vi "Obtain Request Events.vi"(8 "error in":errorcluster, 10 "Create New? (F)":bool) -> (0 "error out":errorcluster, 2 "Data Viewer Request Events":T1)   [LabVIEW 2020, in "Data Viewer.lvlib"]
doc: "This VI Obtains/Creates the Requests events that will be used for other modules to communicate with the module that owns this VI. These Requests events will be accessed only via Public API methods for this module.\n\n<b>NOTE</b>: The contents of this VI are automatically generated and modified by the <b>Tools > DQMH Consortium > DQMH</b> utilities. Consider using those utilities instead of making your own modifications to this VI.\n_____\nBased on DQMH Project Template 7.0.1.1316."
uses:
  Data Viewer.lvlib
  Request Events--cluster.ctl
  Stop Argument--cluster.ctl
  Show Panel Argument--cluster.ctl
  Hide Panel Argument--cluster.ctl
  Show Diagram Argument--cluster.ctl
  Get Module Execution Status Argument--cluster.ctl
  Window Resize Argument--cluster.ctl
  Open File Argument--cluster.ctl
  Draw Plot Argument--cluster.ctl
  Set YScale Argument--cluster.ctl
  Update Curve Color Argument--cluster.ctl
  Show Value Argument--cluster.ctl
  <vilib>/Utility/miscctls.llb/LVPoint32TypeDef.ctl
  Menu Action Argument--cluster.ctl
  Update Filter Arguments Argument--cluster.ctl
  Filte Data Argument--cluster.ctl
  Restore Data Argument--cluster.ctl
  Cut Half Data Argument--cluster.ctl
  Select Point Argument--cluster.ctl
  Open Linear Measurement Argument--cluster.ctl
  Linear Measurement Close Argument--cluster.ctl
  Scale List Menu Action Argument--cluster.ctl
  Update Scale List Argument--cluster.ctl
  Initialize Plot List Argument--cluster.ctl
  Load Plot Argument--cluster.ctl
  Unload Plot Argument--cluster.ctl
  Show Hide Scale Argument--cluster.ctl
  Add Default Scale Argument--cluster.ctl
  Update Plot List Argument--cluster.ctl
  Add Virtual Cruve Argument--cluster.ctl
  Edit Curve Argument--cluster.ctl
panel:
  # "NOTE: The contents of this VI are automatically generated and modified by the Tools > DQMH Consortium > DQMH utilities. Consider using those utilities instead of making your own modifications to this VI."
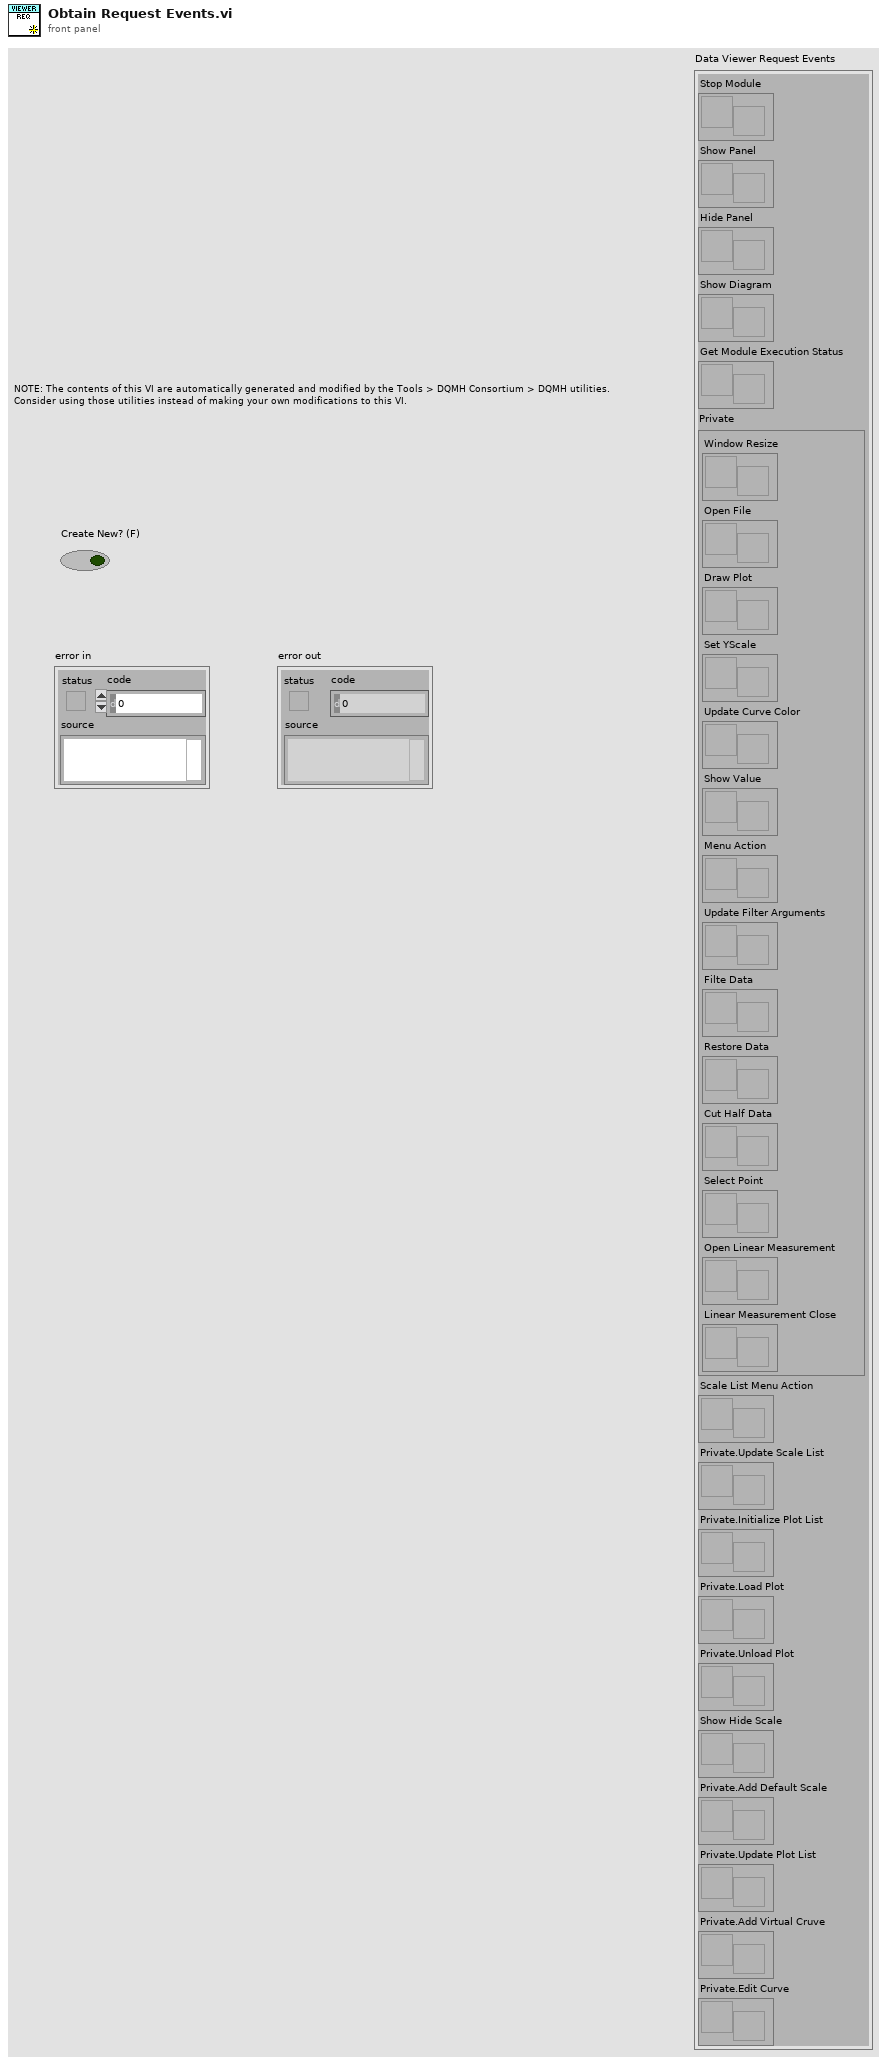
[diagram p1: front panel]
types:
  T1 = typedef "Data Viewer.lvlib/Request Events--cluster.ctl" = cluster{"Stop Module":refnum<user-event>, "Show Panel":refnum<user-event>, "Hide Panel":refnum<user-event>, "Show Diagram":refnum<user-event>, "Get Module Execution Status":refnum<user-event>, "Private":cluster{"Window Resize":refnum<user-event>, "Open File":refnum<user-event>, "Draw Plot":refnum<user-event>, "Set YScale":refnum<user-event>, "Update Curve Color":refnum<user-event>, "Show Value":refnum<user-event>, "Menu Action":refnum<user-event>, "Update Filter Arguments":refnum<user-event>, "Filte Data":refnum<user-event>, "Restore Data":refnum<user-event>, "Cut Half Data":refnum<user-event>, "Select Point":refnum<user-event>, "Open Linear Measurement":refnum<user-event>, "Linear Measurement Close":refnum<user-event>}, "Scale List Menu Action":refnum<user-event>, "Private.Update Scale List":refnum<user-event>, "Private.Initialize Plot List":refnum<user-event>, "Private.Load Plot":refnum<user-event>, "Private.Unload Plot":refnum<user-event>, "Show Hide Scale":refnum<user-event>, "Private.Add Default Scale":refnum<user-event>, "Private.Update Plot List":refnum<user-event>, "Private.Add Virtual Cruve":refnum<user-event>, "Private.Edit Curve":refnum<user-event>}
  T2 = typedef "Data Viewer.lvlib/Edit Curve Argument--cluster.ctl" = cluster{"Module ID":i32, "Plot Index":i32}
  T3 = typedef "Data Viewer.lvlib/Add Virtual Cruve Argument--cluster.ctl" = cluster{"Module ID":i32, "Boolean":bool}
  T4 = typedef "Data Viewer.lvlib/Update Plot List Argument--cluster.ctl" = cluster{"Module ID":i32, "曲线列表":cluster{"Name":string, "Scale":u16, "Color":u32, "Visible":bool, "Peak Line":bool}[]}
  T5 = typedef "Data Viewer.lvlib/Add Default Scale Argument--cluster.ctl" = cluster{"Module ID":i32, "Boolean":bool}
  T6 = typedef "Data Viewer.lvlib/Show Hide Scale Argument--cluster.ctl" = cluster{"Module ID":i32, "Scale Index":i32, "Visible":bool}
  T7 = typedef "Data Viewer.lvlib/Unload Plot Argument--cluster.ctl" = cluster{"Module ID":i32, "Plot Index":i32}
  T8 = typedef "Data Viewer.lvlib/Load Plot Argument--cluster.ctl" = cluster{"Module ID":i32, "Plot Index":i32}
  T9 = typedef "Data Viewer.lvlib/Initialize Plot List Argument--cluster.ctl" = cluster{"Module ID":i32, "Boolean":bool}
  T10 = typedef "Data Viewer.lvlib/Update Scale List Argument--cluster.ctl" = cluster{"Module ID":i32, "Boolean":bool}
  T11 = typedef "Data Viewer.lvlib/Scale List Menu Action Argument--cluster.ctl" = cluster{"Module ID":i32, "ItemTag ":string, "Scale Index":i32}
  T12 = typedef "Data Viewer.lvlib/Linear Measurement Close Argument--cluster.ctl" = cluster{"Module ID":i32, "Linear Measurement Module ID":i32}
  T13 = typedef "Data Viewer.lvlib/Open Linear Measurement Argument--cluster.ctl" = cluster{"Module ID":i32, "Linear Measurement Module ID":i32}
  T14 = typedef "Data Viewer.lvlib/Select Point Argument--cluster.ctl" = cluster{"Module ID":i32, "布尔":bool}
  T15 = typedef "Data Viewer.lvlib/Cut Half Data Argument--cluster.ctl" = cluster{"Module ID":i32, "布尔":bool}
  T16 = typedef "Data Viewer.lvlib/Restore Data Argument--cluster.ctl" = cluster{"Module ID":i32, "布尔":bool}
  T17 = typedef "Data Viewer.lvlib/Filte Data Argument--cluster.ctl" = cluster{"Module ID":i32, "布尔":bool}
  T18 = typedef "Data Viewer.lvlib/Update Filter Arguments Argument--cluster.ctl" = cluster{"Module ID":i32, "布尔":bool}
  T19 = typedef "Data Viewer.lvlib/Menu Action Argument--cluster.ctl" = cluster{"Module ID":i32, "项标识符":string}
  T20 = typedef "Data Viewer.lvlib/Show Value Argument--cluster.ctl" = cluster{"Module ID":i32, "坐标":T21}
  T21 = typedef "LVPoint32TypeDef.ctl" = cluster{"Horizontal":i32, "Vertical":i32}
  T22 = typedef "Data Viewer.lvlib/Update Curve Color Argument--cluster.ctl" = cluster{"Module ID":i32, "布尔":bool}
  T23 = typedef "Data Viewer.lvlib/Set YScale Argument--cluster.ctl" = cluster{"Module ID":i32, "布尔":bool}
  T24 = typedef "Data Viewer.lvlib/Draw Plot Argument--cluster.ctl" = cluster{"Module ID":i32, "布尔":bool}
  T25 = typedef "Data Viewer.lvlib/Open File Argument--cluster.ctl" = cluster{"Module ID":i32, "布尔":bool}
  T26 = typedef "Data Viewer.lvlib/Window Resize Argument--cluster.ctl" = cluster{"Module ID":i32, "布尔":bool}
  T27 = typedef "Data Viewer.lvlib/Get Module Execution Status Argument--cluster.ctl" = cluster{"Module ID":i32, "Running?":bool}
  T28 = typedef "Data Viewer.lvlib/Show Diagram Argument--cluster.ctl" = cluster{"Module ID":i32, "Debug?":bool}
  T29 = typedef "Data Viewer.lvlib/Show Panel Argument--cluster.ctl" = cluster{"Module ID":i32, "Show Panel?":bool}
  T30 = typedef "Data Viewer.lvlib/Hide Panel Argument--cluster.ctl" = cluster{"Module ID":i32, "Hide Panel?":bool}
  T31 = typedef "Data Viewer.lvlib/Stop Argument--cluster.ctl" = cluster{"Module ID":i32, "Origin":string, "Exit via Stop Module Req?":bool, "Wait for Module to stop?":bool}
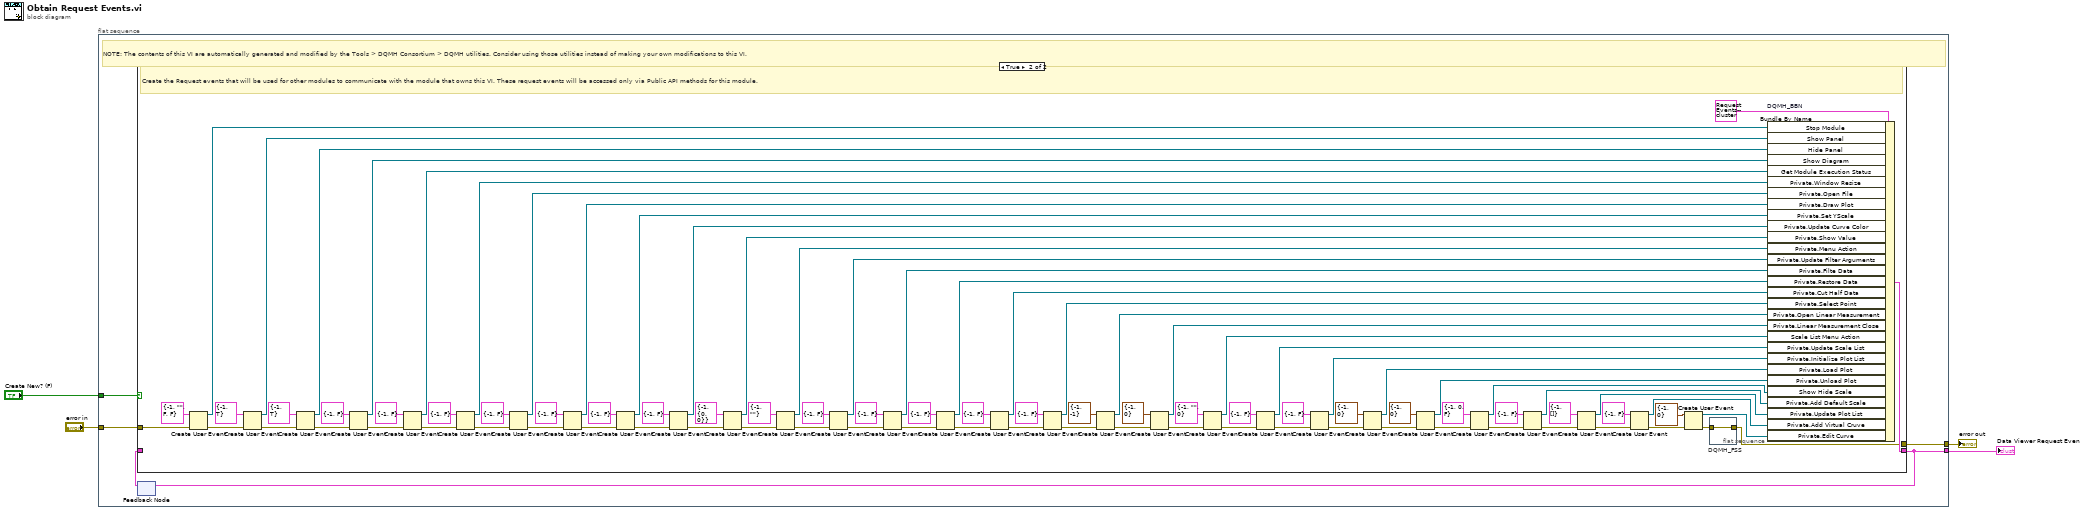
[diagram p0: block diagram]
diagram:
  n1 = flat-sequence {
    tunnel: [w9] -> w4
    tunnel: "error in" -> [w8]
    tunnel: [w6] -> w2
    tunnel: "Create New? (F)" -> [w5]
    frame #0 {
      # "NOTE: The contents of this VI are automatically generated and modified by the Tools > DQMH Consortium > DQMH utilities. Consider using those utilities instead of making your own modifications to this VI."
      n2 = feedback #1() -> (w7:T1)  [unwired: 1 in]
      n3 = case shown="True" w5 {
        tunnel: [w10 w90] -> w9
        tunnel: w8 -> [w10 w102]
        tunnel: [w11 w99] -> w6
        tunnel: w7 -> [w11 _]
        frame False {
        }
        frame True {
          # "Create the Request events that will be used for other modules to communicate with the module that owns this VI. These request events will be accessed only via Public API methods for this module."
          n4 = Create User Event(user event datatype=T31 {"Module ID"=-1, "Origin"="", "Exit via Stop Module Req?"=FALSE, "Wait for Module to stop?"=FALSE} ("Stop Argument"), error in=w102) -> (user event=w100:refnum<user-event>, error out=w97:errorcluster)
          n5 = Create User Event(user event datatype=T29 {"Module ID"=-1, "Show Panel?"=TRUE} ("Show Panel Argument"), error in=w97) -> (user event=w96:refnum<user-event>, error out=w94:errorcluster)
          n6 = Create User Event(user event datatype=T30 {"Module ID"=-1, "Hide Panel?"=TRUE} ("Hide Panel"), error in=w94) -> (user event=w93:refnum<user-event>, error out=w92:errorcluster)
          n7 = Create User Event(user event datatype=T28 {"Module ID"=-1, "Debug?"=FALSE} ("Show Diagram Argument"), error in=w92) -> (user event=w88:refnum<user-event>, error out=w89:errorcluster)
          n8 = Create User Event(user event datatype=T27 {"Module ID"=-1, "Running?"=FALSE} ("Get Module Execution Status Argument"), error in=w89) -> (user event=w85:refnum<user-event>, error out=w86:errorcluster)
          n9 = Create User Event(user event datatype=T26 {"Module ID"=-1, "布尔"=FALSE} ("Window Resize Argument"), error in=w86) -> (user event=w82:refnum<user-event>, error out=w83:errorcluster)
          n10 = Create User Event(user event datatype=T25 {"Module ID"=-1, "布尔"=FALSE} ("Open File Argument"), error in=w83) -> (user event=w79:refnum<user-event>, error out=w80:errorcluster)
          n11 = Create User Event(user event datatype=T24 {"Module ID"=-1, "布尔"=FALSE} ("Draw Plot Argument"), error in=w80) -> (user event=w76:refnum<user-event>, error out=w77:errorcluster)
          n12 = Create User Event(user event datatype=T23 {"Module ID"=-1, "布尔"=FALSE} ("Set YScale Argument"), error in=w77) -> (user event=w73:refnum<user-event>, error out=w74:errorcluster)
          n13 = Create User Event(user event datatype=T22 {"Module ID"=-1, "布尔"=FALSE} ("Update Curve Color Argument"), error in=w74) -> (user event=w70:refnum<user-event>, error out=w71:errorcluster)
          n14 = Create User Event(user event datatype=T20 {"Module ID"=-1, "坐标"={"Horizontal"=0, "Vertical"=0}} ("Show Value Argument"), error in=w71) -> (user event=w67:refnum<user-event>, error out=w68:errorcluster)
          n15 = Create User Event(user event datatype=T19 {"Module ID"=-1, "项标识符"=""} ("Menu Action Argument"), error in=w68) -> (user event=w64:refnum<user-event>, error out=w65:errorcluster)
          n16 = Create User Event(user event datatype=T18 {"Module ID"=-1, "布尔"=FALSE} ("Update Filter Arguments Argument"), error in=w65) -> (user event=w61:refnum<user-event>, error out=w62:errorcluster)
          n17 = Create User Event(user event datatype=T17 {"Module ID"=-1, "布尔"=FALSE} ("Filte Data Argument"), error in=w62) -> (user event=w58:refnum<user-event>, error out=w59:errorcluster)
          n18 = Create User Event(user event datatype=T16 {"Module ID"=-1, "布尔"=FALSE} ("Restore Data Argument"), error in=w59) -> (user event=w55:refnum<user-event>, error out=w56:errorcluster)
          n19 = Create User Event(user event datatype=T15 {"Module ID"=-1, "布尔"=FALSE} ("Cut Half Data Argument"), error in=w56) -> (user event=w52:refnum<user-event>, error out=w53:errorcluster)
          n20 = Create User Event(user event datatype=T14 {"Module ID"=-1, "布尔"=FALSE} ("Select Point Argument"), error in=w53) -> (user event=w49:refnum<user-event>, error out=w50:errorcluster)
          n21 = Create User Event(user event datatype=T13 {"Module ID"=-1, "Linear Measurement Module ID"=-1} ("Open Linear Measurement Argument"), error in=w50) -> (user event=w46:refnum<user-event>, error out=w47:errorcluster)
          n22 = Create User Event(user event datatype=T12 {"Module ID"=-1, "Linear Measurement Module ID"=0} ("Linear Measurement Close Argument"), error in=w47) -> (user event=w43:refnum<user-event>, error out=w44:errorcluster)
          n23 = Create User Event(user event datatype=T11 {"Module ID"=-1, "ItemTag "="", "Scale Index"=0} ("Scale List Menu Action Argument"), error in=w44) -> (user event=w40:refnum<user-event>, error out=w41:errorcluster)
          n24 = Create User Event(user event datatype=T10 {"Module ID"=-1, "Boolean"=FALSE} ("Update Scale List Argument"), error in=w41) -> (user event=w37:refnum<user-event>, error out=w38:errorcluster)
          n25 = Create User Event(user event datatype=T9 {"Module ID"=-1, "Boolean"=FALSE} ("Initialize Plot List Argument"), error in=w38) -> (user event=w34:refnum<user-event>, error out=w35:errorcluster)
          n26 = Create User Event(user event datatype=T8 {"Module ID"=-1, "Plot Index"=0} ("Load Plot Argument"), error in=w35) -> (user event=w31:refnum<user-event>, error out=w32:errorcluster)
          n27 = Create User Event(user event datatype=T7 {"Module ID"=-1, "Plot Index"=0} ("Unload Plot Argument"), error in=w32) -> (user event=w28:refnum<user-event>, error out=w29:errorcluster)
          n28 = Create User Event(user event datatype=T6 {"Module ID"=-1, "Scale Index"=0, "Visible"=FALSE} ("Show Hide Scale Argument"), error in=w29) -> (user event=w25:refnum<user-event>, error out=w26:errorcluster)
          n29 = Create User Event(user event datatype=T5 {"Module ID"=-1, "Boolean"=FALSE} ("Add Default Scale Argument"), error in=w26) -> (user event=w22:refnum<user-event>, error out=w23:errorcluster)
          n30 = Create User Event(user event datatype=T4 {"Module ID"=-1, "曲线列表"=[]} ("Update Plot List Argument"), error in=w23) -> (user event=w19:refnum<user-event>, error out=w20:errorcluster)
          n31 = Create User Event(user event datatype=T3 {"Module ID"=-1, "Boolean"=FALSE} ("Add Virtual Cruve Argument"), error in=w20) -> (user event=w16:refnum<user-event>, error out=w17:errorcluster)
          n32 = Create User Event(user event datatype=T2 {"Module ID"=-1, "Plot Index"=0} ("Edit Curve Argument"), error in=w17) -> (user event=w13:refnum<user-event>, error out=w14:errorcluster)
          n33 = flat-sequence "DQMH_FSS" {
            tunnel: w14 -> [w103]
            tunnel: [w103] -> w90
            frame #0 {
            }
          }
          n34 = Bundle By Name "DQMH_BBN"(cluster=T1 {"Stop Module"=refnum, "Show Panel"=refnum, "Hide Panel"=refnum, "Show Diagram"=refnum, "Get Module Execution Status"=refnum, "Private"={"Window Resize"=refnum, "Open File"=refnum, "Draw Plot"=refnum, "Set YScale"=refnum, "Update Curve Color"=refnum, "Show Value"=refnum, "Menu Action"=refnum, "Update Filter Arguments"=refnum, "Filte Data"=refnum, "Restore Data"=refnum, "Cut Half Data"=refnum, "Select Point"=refnum, "Open Linear Measurement"=refnum, "Linear Measurement Close"=refnum}, "Scale List Menu Action"=refnum, "Private.Update Scale List"=refnum, "Private.Initialize Plot List"=refnum, "Private.Load Plot"=refnum, "Private.Unload Plot"=refnum, "Show Hide Scale"=refnum, "Private.Add Default Scale"=refnum, "Private.Update Plot List"=refnum, "Private.Add Virtual Cruve"=refnum, "Private.Edit Curve"=refnum} ("output cluster"), "Stop Module"=w100, "Show Panel"=w96, "Hide Panel"=w93, "Show Diagram"=w88, "Get Module Execution Status"=w85, "Private.Window Resize"=w82, "Private.Open File"=w79, "Private.Draw Plot"=w76, "Private.Set YScale"=w73, "Private.Update Curve Color"=w70, "Private.Show Value"=w67, "Private.Menu Action"=w64, "Private.Update Filter Arguments"=w61, "Private.Filte Data"=w58, "Private.Restore Data"=w55, "Private.Cut Half Data"=w52, "Private.Select Point"=w49, "Private.Open Linear Measurement"=w46, "Private.Linear Measurement Close"=w43, "Scale List Menu Action"=w40, "Private.Update Scale List"=w37, "Private.Initialize Plot List"=w34, "Private.Load Plot"=w31, "Private.Unload Plot"=w28, "Show Hide Scale"=w25, "Private.Add Default Scale"=w22, "Private.Update Plot List"=w19, "Private.Add Virtual Cruve"=w16, "Private.Edit Curve"=w13) -> (w99:T1)
        }
      }
      n35 = feedback-in #1(w6) -> ()
    }
  }
  "Data Viewer Request Events" <- w2
  "error out" <- w4
